vi "Signal-simulator.vi"(9 "phases [deg]":dbl[](array[numeric])=[0.0, 90.0, 270.0], 10 "amplitudes":dbl[](array[numeric])=[1.0, 1.0, 1.0], 11 "frequencies [Hz]":dbl[](array[numeric])=[100.0, 200.0, 300.0]) -> (0 "error out":errorcluster, 3 "output waveform":waveform(dbl))   [LabVIEW 2026, in "Unit-Test.lvlib"]
uses:
  Unit-Test.lvlib
  <vilib>/addons/_NISVFA/_Generation/Signal Generation/SV Multitone/Configure Multitone (Custom).vi
  <vilib>/addons/_NISVFA/_Generation/Signal Generation/SV Multitone/SV Multitone.lvclass
  <vilib>/addons/_NISVFA/_Generation/Signal Generation/SV Signal/SV Signal.lvclass
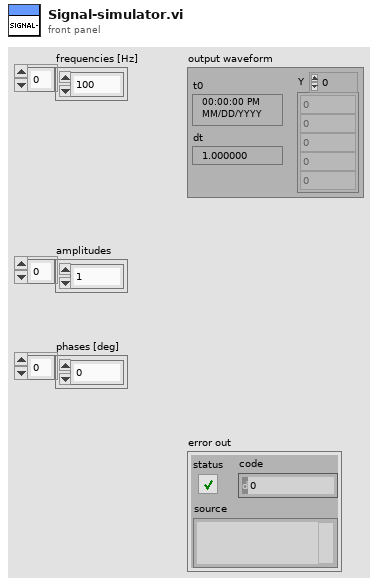
[diagram p1: front panel]
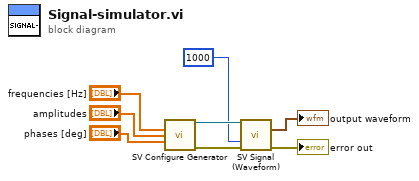
[diagram p0: block diagram]
diagram:
  n1 = call-poly <vilib>:"SV Configure Generator.vi"("frequencies [Hz]"="frequencies [Hz]", "amplitudes"="amplitudes", "phases [deg]"="phases [deg]") -> ("signal configuration"=w4:refnum<class "SV Multitone.lvclass">, "error out"=w2:errorcluster)  [unwired: 10 in, 1 out]
  n2 = call-dynamic "SV Signal (Waveform).vi"("signal configuration"=w4, "samples"=1000, "error in (no error)"=w2) -> ("output waveform"=→"output waveform":waveform(dbl), "error out"=→"error out":errorcluster)  [unwired: 7 in, 4 out]
